vi "VIH Platform - LabVIEW - Open VI Without Refees (2013).vi"(8 "error in":errorcluster, 9 "options":i32 format="%.0x", 11 "VI Path":path) -> (0 "error out":errorcluster, 3 "VI Reference":refnum<vi>, 5 "Tmp App Refnum":refnum<vi>)   [LabVIEW 2014]
doc: "::: VI Helpeks :::\nCopyright (c) 2000-2026 Konstantin Shifershteyn. All rights reserved."
panel:
  # "VI Helpeks\nCopyright (c) 2012-2026 Konstantin Shifershteyn"
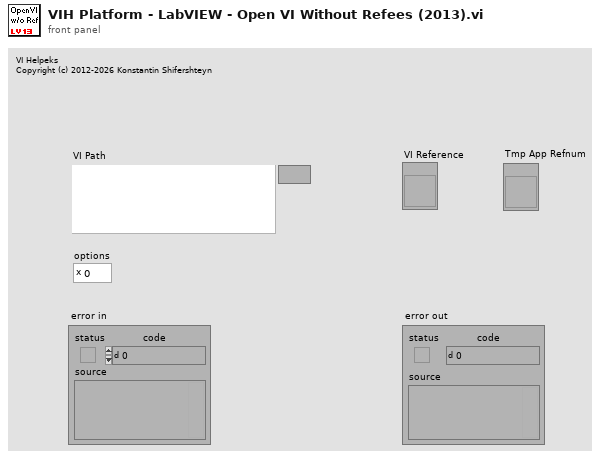
[diagram p1: front panel]
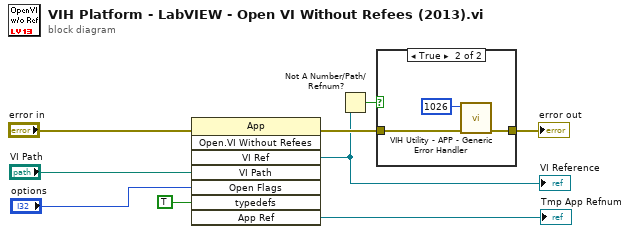
[diagram p0: block diagram]
diagram:
  n1 = invoke class="App" method="Open.VI Without Refees"(error in="error in", "VI Path"="VI Path", "Open Flags"="options", "typedefs"=TRUE) -> (error out=w5:errorcluster, "VI Ref"=w3:refnum<vi>, "App Ref"=→"Tmp App Refnum":refnum<vi>)  [unwired: 4 in, 5 out]
  "VI Reference" <- w3
  n2 = Not A Number/Path/Refnum?(number/path/refnum=w3) -> (NaN/Path/Refnum?=w2:bool)
  n3 = case shown="True" w2 {
    tunnel: w5 -> [w10 w13]
    tunnel: [w10 w12] -> w4
    frame False {
    }
    frame True {
      n4 = call "VIH Utility - APP - Generic Error Handler.vi"("error in"=w13, "error code"=1026) -> ("error out"=w12:errorcluster)  [unwired: 8 in, 1 out]
    }
  }
  "error out" <- w4
